vi "Check Upgrade.vi"(8 "error in (no error)":errorcluster, 10 "Request":refnum<class "Request.lvclass">) -> (0 "error out":errorcluster, 1 "Is WS Upgrade":bool, 2 "Response":refnum<class "WebSocketUpgradeResponse.lvclass">)   [LabVIEW 2020, in "HTTP Server.lvlib" / "WebSocket Client.lvclass"]
uses:
  WebSocket Client.lvclass
  WebSocketUpgradeResponse/WebSocketUpgradeResponse.lvclass
  lv-http-util/HTTP Utils/Method.ctl
  WebSocket Client.lvclass/WebSocket Client.ctl
  lv-http-util/HTTP Utils/Request/Request.lvclass/Request.ctl
  lv-http-util/HTTP Utils/Request/Request.lvclass
  lv-http-util/HTTP Utils/HTTP Utils.lvlib
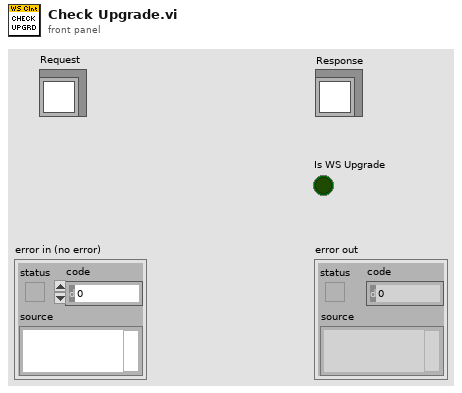
[diagram p1: front panel]
types:
  T1 = typedef "HTTP Utils.lvlib/Method.ctl" = enum16{"GET", "HEAD", "POST", "PUT", "DELETE", "CONNECT", "OPTIONS", "TRACE", "PATCH"}
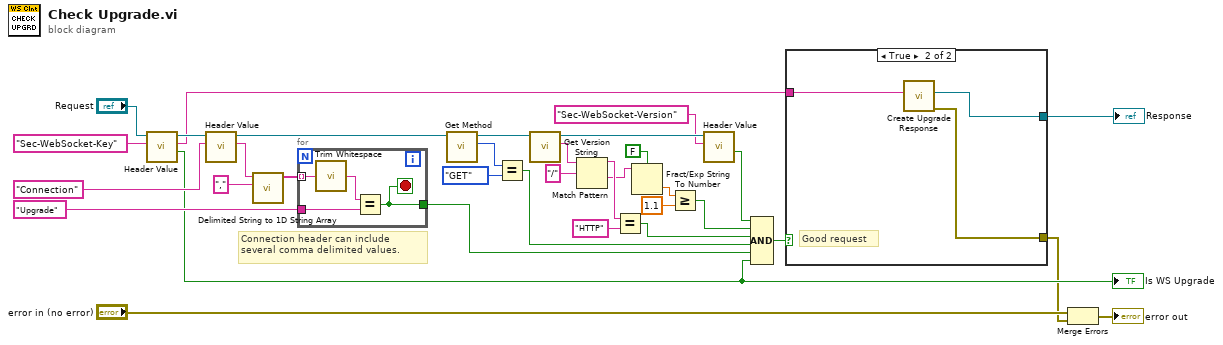
[diagram p0: block diagram]
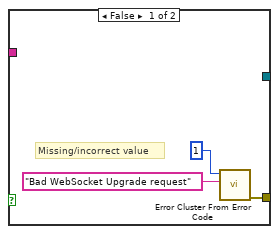
[diagram p2: hidden frame]
diagram:
  # "Connection header can include several comma delimited values."
  n1 = call "Header Value.vi"("Header"="Sec-WebSocket-Key", "Request in"="Request") -> ("Exists"=w6:bool, "Value"=w3:string, "Request out"=w32:refnum<class "Request.lvclass">)  [unwired: 6 in, 1 out]
  "Is WS Upgrade" <- w6
  n2 = call "Header Value.vi"("Header"="Connection", "Request in"=w32) -> ("Value"=w9:string, "Request out"=w28:refnum<class "Request.lvclass">)  [unwired: 6 in, 2 out]
  n3 = call <vilib>:"Delimited String to 1D String Array.vi"("delimiter"=",", "delimited string"=w9) -> ("string array"=w7:string[])  [unwired: 9 in]
  n4 = for {
    tunnel: "Upgrade" -> [w38]
    tunnel: [w35] -> w29
    tunnel: w7 -> [w37] mode=indexing
    stop <- w35 stop-if-true
    n5 = call <vilib>:"Trim Whitespace.vi"("string"=w37) -> ("trimmed string"=w36:string)  [unwired: 1 in]
    n6 = Equal?(x=w36, y=w38) -> (x = y?=w35:bool)
  }
  n7 = call "Get Method.vi"("Request in"=w28) -> ("Method"=w27:T1, "Request out"=w25:refnum<class "Request.lvclass">)  [unwired: 8 in, 1 out]
  n8 = Equal?(x=w27, y=Method."GET") -> (x = y?=w24:bool)
  n9 = call "Get Version String.vi"("Request in"=w25) -> ("Version String"=w23:string, "Request out"=w14:refnum<class "Request.lvclass">)  [unwired: 8 in, 1 out]
  n10 = Match Pattern(string=w23, regular expression="/") -> (before substring=w21:string, after substring=w19:string)  [unwired: 1 in, 2 out]
  n11 = Equal?(x=w21, y="HTTP") -> (x = y?=w17:bool)
  n12 = Fract/Exp String To Number(use system decimal point (T)=FALSE, string=w19) -> (number=w18:dbl)  [unwired: 2 in, 1 out]
  n13 = Greater Or Equal?(x=w18, y=1.1) -> (x >= y?=w15:bool)
  n14 = call "Header Value.vi"("Header"="Sec-WebSocket-Version", "Request in"=w14) -> ("Exists"=w12:bool)  [unwired: 6 in, 3 out]
  n15 = Compound Arithmetic op=AND(w12, w15, w17, w24, w29, w6) -> (w11:bool)
  n16 = case shown="True" w11 {
    tunnel: [w39 w43] -> w4
    tunnel: w3 -> [_ w44]
    tunnel: [_ w42] -> w2
    frame False {
      # "Missing/incorrect value"
      n17 = call <vilib>:"Error Cluster From Error Code.vi"("error message (\"\")"="Bad WebSocket Upgrade request" ("error message (\"\")"), "error code (0)"=1) -> ("error out"=w39:errorcluster)  [unwired: 7 in]
    }
    frame True {
      # "Good request"
      n18 = call "Create Upgrade Response.vi"("Sec-WebSocket-Key"=w44) -> ("error out"=w43:errorcluster, "WebSocketUpgradeResponse"=w42:refnum<class "WebSocketUpgradeResponse.lvclass">)  [unwired: 9 in]
    }
  }
  "Response" <- w2
  n19 = Merge Errors("error in (no error)", w4) -> (→"error out":errorcluster)
